vi "theremin.vi"() -> ()   [LabVIEW 2024]
uses:
  <vilib>/Instr/_visa.llb/VISA Configure Serial Port (Instr).vi
panel:
  out "STANDBY":bool
  out "G#":bool
  out "G":bool
  out "F#":bool
  out "F":bool
  out "E":bool
  out "D#":bool
  out "D":bool
  out "C#":bool
  out "C":bool
  out "B":bool
  out "A#":bool
  out "A":bool
  out "Octave 8":bool
  out "Octave 7":bool
  out "Octave 6":bool
  out "Octave 5":bool
  out "Octave 4":bool
  out "Octave 3":bool
  out "Octave 2":bool
  out "Octave 1":bool
  out "Octave 0":bool
  out "Frequency":dbl
  in  "stop":bool
  out "Volume":dbl(knob) scale=0.0..255.0
  out "Pitch":dbl(knob) scale=0.0..1000.0
  in  "VISA resource name":refnum<visa-resource-name>
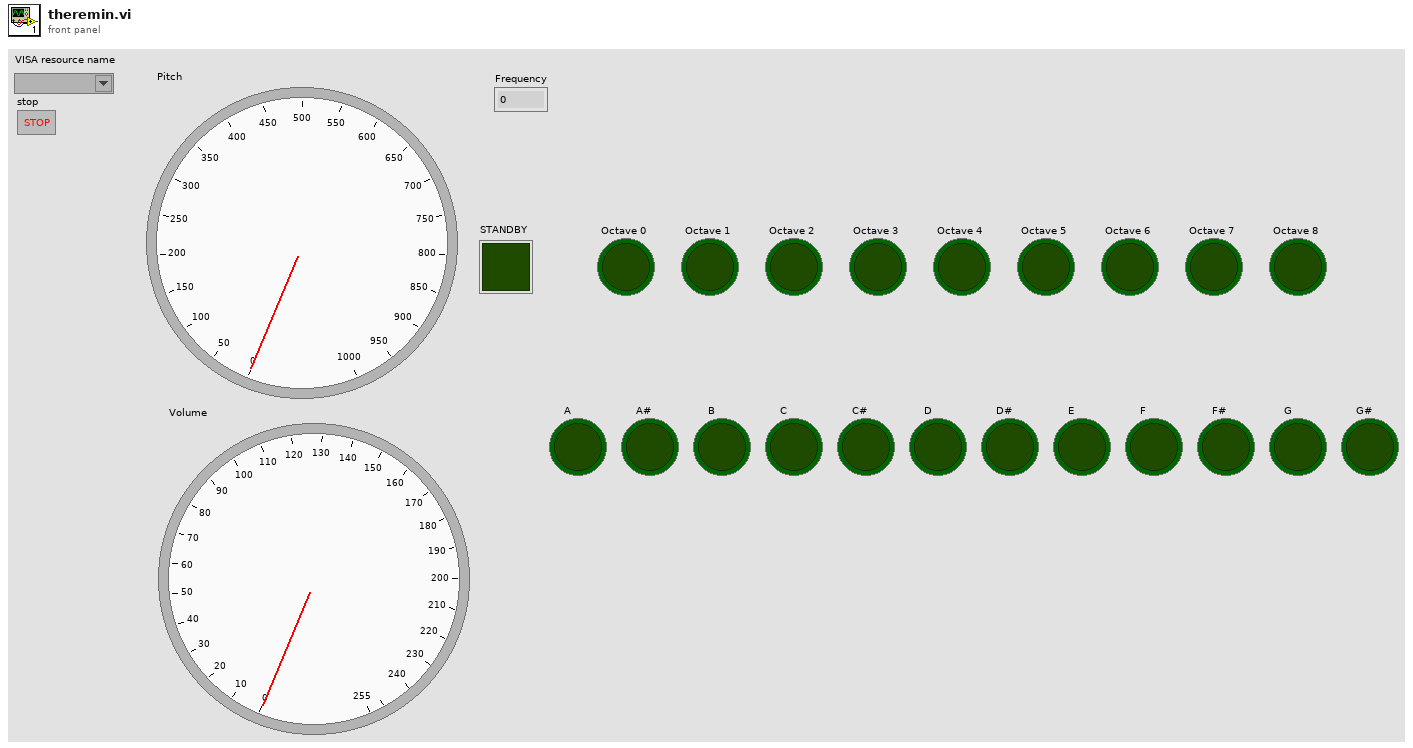
[diagram p1: front panel]
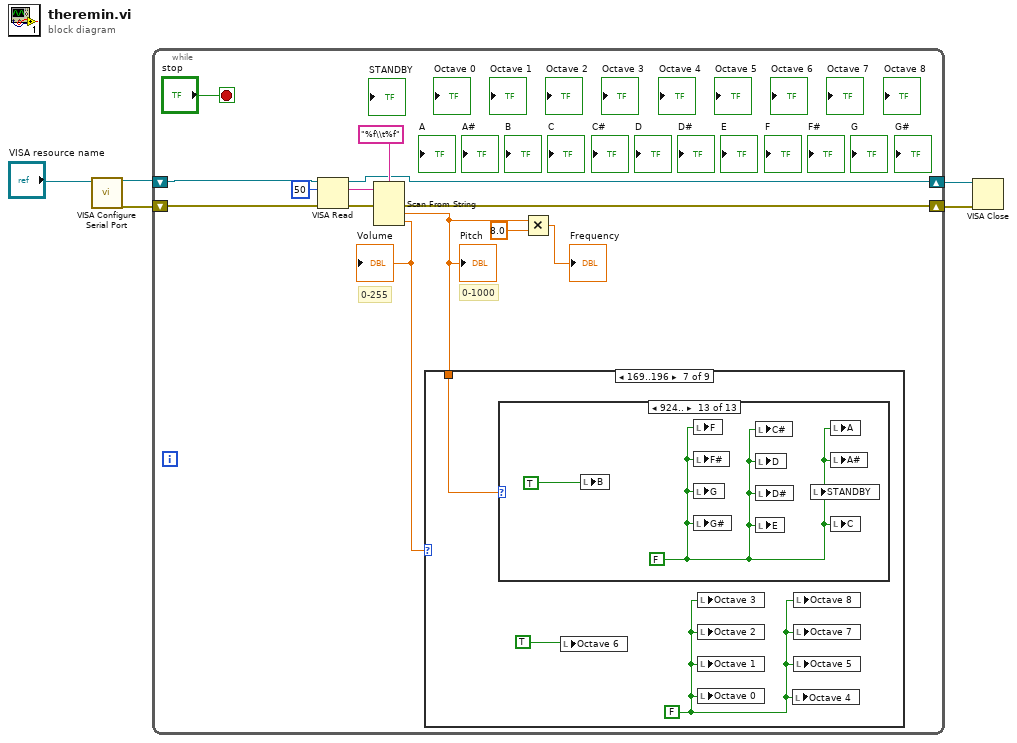
[diagram p0: block diagram]
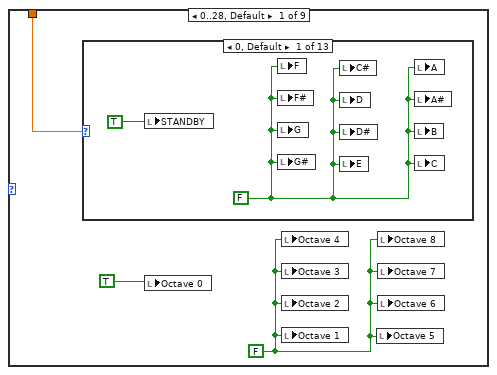
[diagram p2: hidden frame]
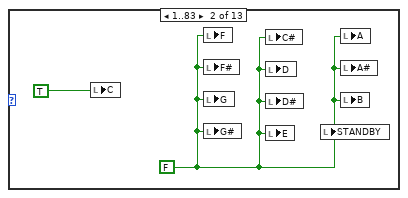
[diagram p3: hidden frame]
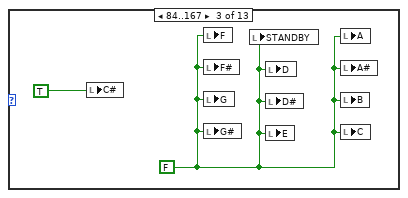
[diagram p4: hidden frame]
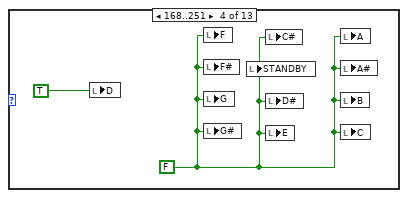
[diagram p5: hidden frame]
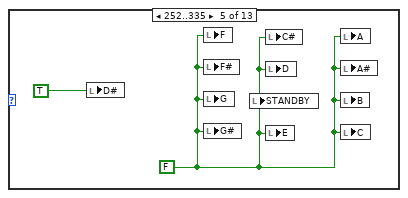
[diagram p6: hidden frame]
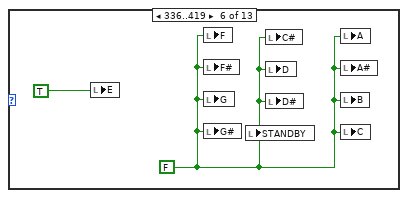
[diagram p7: hidden frame]
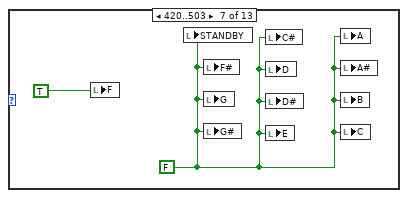
[diagram p8: hidden frame]
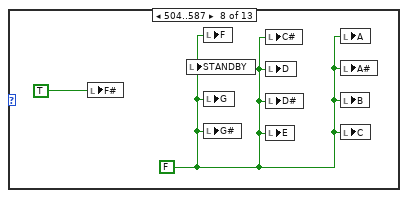
[diagram p9: hidden frame]
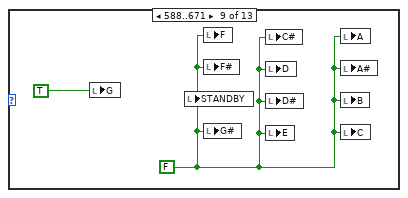
[diagram p10: hidden frame]
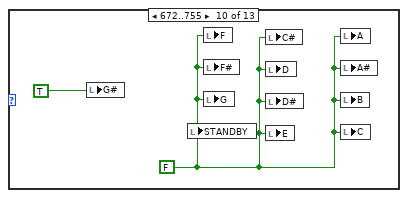
[diagram p11: hidden frame]
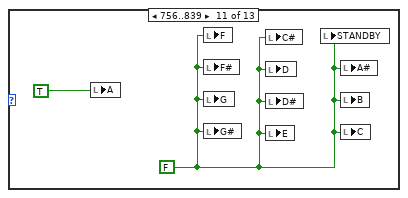
[diagram p12: hidden frame]
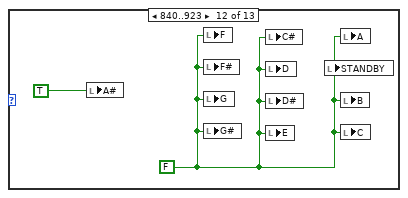
[diagram p13: hidden frame]
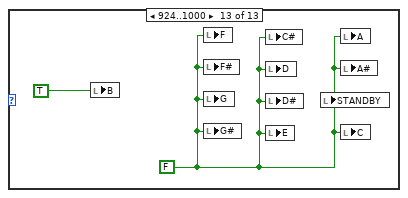
[diagram p14: hidden frame]
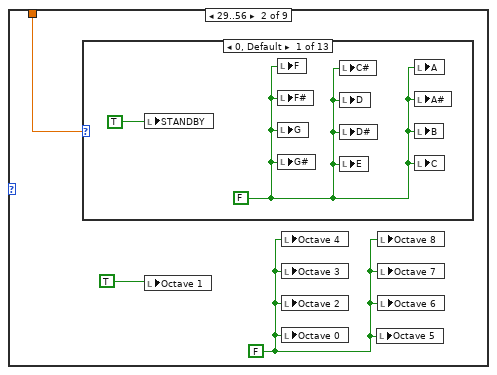
[diagram p15: hidden frame]
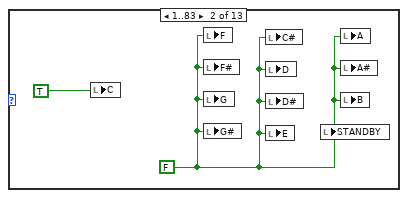
[diagram p16: hidden frame]
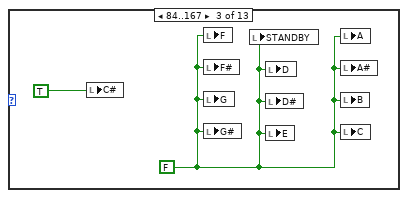
[diagram p17: hidden frame]
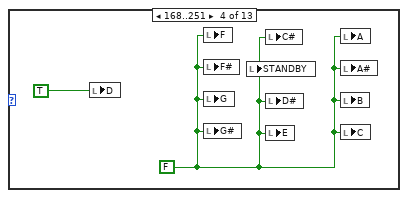
[diagram p18: hidden frame]
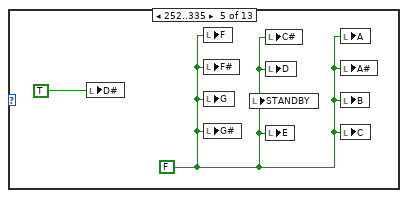
[diagram p19: hidden frame]
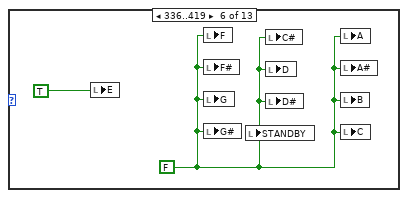
[diagram p20: hidden frame]
diagram:
  n1 = call-poly "VISA Configure Serial Port"("VISA resource name"="VISA resource name") -> ("VISA resource name out"=w3:refnum<visa-resource-name>, "error out"=w2:errorcluster)  [unwired: 13 in]
  n2 = while {
    shift-right: [w15] -> w4
    shift-left: w3 -> [w12]
    shift-right: [w18] -> w5
    shift-left: w2 -> [w13]
    stop <- "stop" stop-if-true
    # "0-1000"
    # "0-255"
    n3 = VISA Read(VISA resource name=w12, byte count=u32 50, error in (no error)=w13) -> (VISA resource name out=w15:refnum<visa-resource-name>, read buffer=w10:string, error out=w14:errorcluster)  [unwired: 1 out]
    n4 = Scan From String(format string="%f\\t%f", input string=w10, error in=w14) -> (error out=w18:errorcluster, output 1=w7:dbl, output 2=w6:dbl)  [unwired: 3 in, 2 out]
    "Pitch" <- w7
    "Volume" <- w6
    n5 = case shown="169..196" w6 {
      tunnel: w7 -> [w21 w50 w79 w108 w137 w166 w195 w224 w253]
      frame 0..28, Default {
        w19 = FALSE
        n6 = case shown="0, Default" w21 {
          frame 0, Default {
            w22 = FALSE
            n7 = local write "STANDBY"(TRUE) -> ()
            n8 = local write "F"(w22) -> ()
            n9 = local write "F#"(w22) -> ()
            n10 = local write "G"(w22) -> ()
            n11 = local write "G#"(w22) -> ()
            n12 = local write "C#"(w22) -> ()
            n13 = local write "D"(w22) -> ()
            n14 = local write "D#"(w22) -> ()
            n15 = local write "E"(w22) -> ()
            n16 = local write "A"(w22) -> ()
            n17 = local write "A#"(w22) -> ()
            n18 = local write "B"(w22) -> ()
            n19 = local write "C"(w22) -> ()
          }
          frame 1..83 {
            w24 = FALSE
            n20 = local write "C"(TRUE) -> ()
            n21 = local write "F"(w24) -> ()
            n22 = local write "F#"(w24) -> ()
            n23 = local write "G"(w24) -> ()
            n24 = local write "G#"(w24) -> ()
            n25 = local write "C#"(w24) -> ()
            n26 = local write "D"(w24) -> ()
            n27 = local write "D#"(w24) -> ()
            n28 = local write "E"(w24) -> ()
            n29 = local write "STANDBY"(w24) -> ()
            n30 = local write "A"(w24) -> ()
            n31 = local write "A#"(w24) -> ()
            n32 = local write "B"(w24) -> ()
          }
          frame 84..167 {
            w26 = FALSE
            n33 = local write "C#"(TRUE) -> ()
            n34 = local write "F"(w26) -> ()
            n35 = local write "F#"(w26) -> ()
            n36 = local write "G"(w26) -> ()
            n37 = local write "G#"(w26) -> ()
            n38 = local write "STANDBY"(w26) -> ()
            n39 = local write "D"(w26) -> ()
            n40 = local write "D#"(w26) -> ()
            n41 = local write "E"(w26) -> ()
            n42 = local write "A"(w26) -> ()
            n43 = local write "A#"(w26) -> ()
            n44 = local write "B"(w26) -> ()
            n45 = local write "C"(w26) -> ()
          }
          frame 168..251 {
            w28 = FALSE
            n46 = local write "D"(TRUE) -> ()
            n47 = local write "F"(w28) -> ()
            n48 = local write "F#"(w28) -> ()
            n49 = local write "G"(w28) -> ()
            n50 = local write "G#"(w28) -> ()
            n51 = local write "STANDBY"(w28) -> ()
            n52 = local write "C#"(w28) -> ()
            n53 = local write "D#"(w28) -> ()
            n54 = local write "E"(w28) -> ()
            n55 = local write "A"(w28) -> ()
            n56 = local write "A#"(w28) -> ()
            n57 = local write "B"(w28) -> ()
            n58 = local write "C"(w28) -> ()
          }
          frame 252..335 {
            w30 = FALSE
            n59 = local write "D#"(TRUE) -> ()
            n60 = local write "F"(w30) -> ()
            n61 = local write "F#"(w30) -> ()
            n62 = local write "G"(w30) -> ()
            n63 = local write "G#"(w30) -> ()
            n64 = local write "STANDBY"(w30) -> ()
            n65 = local write "C#"(w30) -> ()
            n66 = local write "D"(w30) -> ()
            n67 = local write "E"(w30) -> ()
            n68 = local write "A"(w30) -> ()
            n69 = local write "A#"(w30) -> ()
            n70 = local write "B"(w30) -> ()
            n71 = local write "C"(w30) -> ()
          }
          frame 336..419 {
            w32 = FALSE
            n72 = local write "E"(TRUE) -> ()
            n73 = local write "F"(w32) -> ()
            n74 = local write "F#"(w32) -> ()
            n75 = local write "G"(w32) -> ()
            n76 = local write "G#"(w32) -> ()
            n77 = local write "STANDBY"(w32) -> ()
            n78 = local write "C#"(w32) -> ()
            n79 = local write "D"(w32) -> ()
            n80 = local write "D#"(w32) -> ()
            n81 = local write "A"(w32) -> ()
            n82 = local write "A#"(w32) -> ()
            n83 = local write "B"(w32) -> ()
            n84 = local write "C"(w32) -> ()
          }
          frame 420..503 {
            w34 = FALSE
            n85 = local write "F"(TRUE) -> ()
            n86 = local write "STANDBY"(w34) -> ()
            n87 = local write "F#"(w34) -> ()
            n88 = local write "G"(w34) -> ()
            n89 = local write "G#"(w34) -> ()
            n90 = local write "C#"(w34) -> ()
            n91 = local write "D"(w34) -> ()
            n92 = local write "D#"(w34) -> ()
            n93 = local write "E"(w34) -> ()
            n94 = local write "A"(w34) -> ()
            n95 = local write "A#"(w34) -> ()
            n96 = local write "B"(w34) -> ()
            n97 = local write "C"(w34) -> ()
          }
          frame 504..587 {
            w36 = FALSE
            n98 = local write "F#"(TRUE) -> ()
            n99 = local write "STANDBY"(w36) -> ()
            n100 = local write "F"(w36) -> ()
            n101 = local write "G"(w36) -> ()
            n102 = local write "G#"(w36) -> ()
            n103 = local write "C#"(w36) -> ()
            n104 = local write "D"(w36) -> ()
            n105 = local write "D#"(w36) -> ()
            n106 = local write "E"(w36) -> ()
            n107 = local write "A"(w36) -> ()
            n108 = local write "A#"(w36) -> ()
            n109 = local write "B"(w36) -> ()
            n110 = local write "C"(w36) -> ()
          }
          frame 588..671 {
            w38 = FALSE
            n111 = local write "G"(TRUE) -> ()
            n112 = local write "STANDBY"(w38) -> ()
            n113 = local write "F"(w38) -> ()
            n114 = local write "F#"(w38) -> ()
            n115 = local write "G#"(w38) -> ()
            n116 = local write "C#"(w38) -> ()
            n117 = local write "D"(w38) -> ()
            n118 = local write "D#"(w38) -> ()
            n119 = local write "E"(w38) -> ()
            n120 = local write "A"(w38) -> ()
            n121 = local write "A#"(w38) -> ()
            n122 = local write "B"(w38) -> ()
            n123 = local write "C"(w38) -> ()
          }
          frame 672..755 {
            w40 = FALSE
            n124 = local write "G#"(TRUE) -> ()
            n125 = local write "STANDBY"(w40) -> ()
            n126 = local write "F"(w40) -> ()
            n127 = local write "F#"(w40) -> ()
            n128 = local write "G"(w40) -> ()
            n129 = local write "C#"(w40) -> ()
            n130 = local write "D"(w40) -> ()
            n131 = local write "D#"(w40) -> ()
            n132 = local write "E"(w40) -> ()
            n133 = local write "A"(w40) -> ()
            n134 = local write "A#"(w40) -> ()
            n135 = local write "B"(w40) -> ()
            n136 = local write "C"(w40) -> ()
          }
          frame 756..839 {
            w42 = FALSE
            n137 = local write "A"(TRUE) -> ()
            n138 = local write "F"(w42) -> ()
            n139 = local write "F#"(w42) -> ()
            n140 = local write "G"(w42) -> ()
            n141 = local write "G#"(w42) -> ()
            n142 = local write "C#"(w42) -> ()
            n143 = local write "D"(w42) -> ()
            n144 = local write "D#"(w42) -> ()
            n145 = local write "E"(w42) -> ()
            n146 = local write "STANDBY"(w42) -> ()
            n147 = local write "A#"(w42) -> ()
            n148 = local write "B"(w42) -> ()
            n149 = local write "C"(w42) -> ()
          }
          frame 840..923 {
            w44 = FALSE
            n150 = local write "A#"(TRUE) -> ()
            n151 = local write "F"(w44) -> ()
            n152 = local write "F#"(w44) -> ()
            n153 = local write "G"(w44) -> ()
            n154 = local write "G#"(w44) -> ()
            n155 = local write "C#"(w44) -> ()
            n156 = local write "D"(w44) -> ()
            n157 = local write "D#"(w44) -> ()
            n158 = local write "E"(w44) -> ()
            n159 = local write "STANDBY"(w44) -> ()
            n160 = local write "A"(w44) -> ()
            n161 = local write "B"(w44) -> ()
            n162 = local write "C"(w44) -> ()
          }
          frame 924..1000 {
            w46 = FALSE
            n163 = local write "B"(TRUE) -> ()
            n164 = local write "F"(w46) -> ()
            n165 = local write "F#"(w46) -> ()
            n166 = local write "G"(w46) -> ()
            n167 = local write "G#"(w46) -> ()
            n168 = local write "C#"(w46) -> ()
            n169 = local write "D"(w46) -> ()
            n170 = local write "D#"(w46) -> ()
            n171 = local write "E"(w46) -> ()
            n172 = local write "STANDBY"(w46) -> ()
            n173 = local write "A"(w46) -> ()
            n174 = local write "A#"(w46) -> ()
            n175 = local write "C"(w46) -> ()
          }
        }
        n176 = local write "Octave 0"(TRUE) -> ()
        n177 = local write "Octave 4"(w19) -> ()
        n178 = local write "Octave 3"(w19) -> ()
        n179 = local write "Octave 2"(w19) -> ()
        n180 = local write "Octave 1"(w19) -> ()
        n181 = local write "Octave 5"(w19) -> ()
        n182 = local write "Octave 8"(w19) -> ()
        n183 = local write "Octave 7"(w19) -> ()
        n184 = local write "Octave 6"(w19) -> ()
      }
      frame 29..56 {
        w48 = FALSE
        n185 = case shown="0, Default" w50 {
          frame 0, Default {
            w51 = FALSE
            n186 = local write "STANDBY"(TRUE) -> ()
            n187 = local write "F"(w51) -> ()
            n188 = local write "F#"(w51) -> ()
            n189 = local write "G"(w51) -> ()
            n190 = local write "G#"(w51) -> ()
            n191 = local write "C#"(w51) -> ()
            n192 = local write "D"(w51) -> ()
            n193 = local write "D#"(w51) -> ()
            n194 = local write "E"(w51) -> ()
            n195 = local write "A"(w51) -> ()
            n196 = local write "A#"(w51) -> ()
            n197 = local write "B"(w51) -> ()
            n198 = local write "C"(w51) -> ()
          }
          frame 1..83 {
            w53 = FALSE
            n199 = local write "C"(TRUE) -> ()
            n200 = local write "F"(w53) -> ()
            n201 = local write "F#"(w53) -> ()
            n202 = local write "G"(w53) -> ()
            n203 = local write "G#"(w53) -> ()
            n204 = local write "C#"(w53) -> ()
            n205 = local write "D"(w53) -> ()
            n206 = local write "D#"(w53) -> ()
            n207 = local write "E"(w53) -> ()
            n208 = local write "STANDBY"(w53) -> ()
            n209 = local write "A"(w53) -> ()
            n210 = local write "A#"(w53) -> ()
            n211 = local write "B"(w53) -> ()
          }
          frame 84..167 {
            w55 = FALSE
            n212 = local write "C#"(TRUE) -> ()
            n213 = local write "F"(w55) -> ()
            n214 = local write "F#"(w55) -> ()
            n215 = local write "G"(w55) -> ()
            n216 = local write "G#"(w55) -> ()
            n217 = local write "STANDBY"(w55) -> ()
            n218 = local write "D"(w55) -> ()
            n219 = local write "D#"(w55) -> ()
            n220 = local write "E"(w55) -> ()
            n221 = local write "A"(w55) -> ()
            n222 = local write "A#"(w55) -> ()
            n223 = local write "B"(w55) -> ()
            n224 = local write "C"(w55) -> ()
          }
          frame 168..251 {
            w57 = FALSE
            n225 = local write "D"(TRUE) -> ()
            n226 = local write "F"(w57) -> ()
            n227 = local write "F#"(w57) -> ()
            n228 = local write "G"(w57) -> ()
            n229 = local write "G#"(w57) -> ()
            n230 = local write "STANDBY"(w57) -> ()
            n231 = local write "C#"(w57) -> ()
            n232 = local write "D#"(w57) -> ()
            n233 = local write "E"(w57) -> ()
            n234 = local write "A"(w57) -> ()
            n235 = local write "A#"(w57) -> ()
            n236 = local write "B"(w57) -> ()
            n237 = local write "C"(w57) -> ()
          }
          frame 252..335 {
            w59 = FALSE
            n238 = local write "D#"(TRUE) -> ()
            n239 = local write "F"(w59) -> ()
            n240 = local write "F#"(w59) -> ()
            n241 = local write "G"(w59) -> ()
            n242 = local write "G#"(w59) -> ()
            n243 = local write "STANDBY"(w59) -> ()
            n244 = local write "C#"(w59) -> ()
            n245 = local write "D"(w59) -> ()
            n246 = local write "E"(w59) -> ()
            n247 = local write "A"(w59) -> ()
            n248 = local write "A#"(w59) -> ()
            n249 = local write "B"(w59) -> ()
            n250 = local write "C"(w59) -> ()
          }
          frame 336..419 {
            w61 = FALSE
            n251 = local write "E"(TRUE) -> ()
            n252 = local write "F"(w61) -> ()
            n253 = local write "F#"(w61) -> ()
            n254 = local write "G"(w61) -> ()
            n255 = local write "G#"(w61) -> ()
            n256 = local write "STANDBY"(w61) -> ()
            n257 = local write "C#"(w61) -> ()
            n258 = local write "D"(w61) -> ()
            n259 = local write "D#"(w61) -> ()
            n260 = local write "A"(w61) -> ()
            n261 = local write "A#"(w61) -> ()
            n262 = local write "B"(w61) -> ()
            n263 = local write "C"(w61) -> ()
          }
          frame 420..503 {
            w63 = FALSE
            n264 = local write "F"(TRUE) -> ()
            n265 = local write "STANDBY"(w63) -> ()
            n266 = local write "F#"(w63) -> ()
            n267 = local write "G"(w63) -> ()
            n268 = local write "G#"(w63) -> ()
            n269 = local write "C#"(w63) -> ()
            n270 = local write "D"(w63) -> ()
            n271 = local write "D#"(w63) -> ()
            n272 = local write "E"(w63) -> ()
            n273 = local write "A"(w63) -> ()
            n274 = local write "A#"(w63) -> ()
            n275 = local write "B"(w63) -> ()
            n276 = local write "C"(w63) -> ()
          }
          frame 504..587 {
            w65 = FALSE
            n277 = local write "F#"(TRUE) -> ()
            n278 = local write "STANDBY"(w65) -> ()
            n279 = local write "F"(w65) -> ()
            n280 = local write "G"(w65) -> ()
            n281 = local write "G#"(w65) -> ()
            n282 = local write "C#"(w65) -> ()
            n283 = local write "D"(w65) -> ()
            n284 = local write "D#"(w65) -> ()
            n285 = local write "E"(w65) -> ()
            n286 = local write "A"(w65) -> ()
            n287 = local write "A#"(w65) -> ()
            n288 = local write "B"(w65) -> ()
            n289 = local write "C"(w65) -> ()
          }
          frame 588..671 {
            w67 = FALSE
            n290 = local write "G"(TRUE) -> ()
            n291 = local write "STANDBY"(w67) -> ()
            n292 = local write "F"(w67) -> ()
            n293 = local write "F#"(w67) -> ()
            n294 = local write "G#"(w67) -> ()
            n295 = local write "C#"(w67) -> ()
            n296 = local write "D"(w67) -> ()
            n297 = local write "D#"(w67) -> ()
            n298 = local write "E"(w67) -> ()
            n299 = local write "A"(w67) -> ()
            n300 = local write "A#"(w67) -> ()
            n301 = local write "B"(w67) -> ()
            n302 = local write "C"(w67) -> ()
          }
          frame 672..755 {
            w69 = FALSE
            n303 = local write "G#"(TRUE) -> ()
            n304 = local write "STANDBY"(w69) -> ()
            n305 = local write "F"(w69) -> ()
            n306 = local write "F#"(w69) -> ()
            n307 = local write "G"(w69) -> ()
            n308 = local write "C#"(w69) -> ()
            n309 = local write "D"(w69) -> ()
            n310 = local write "D#"(w69) -> ()
            n311 = local write "E"(w69) -> ()
            n312 = local write "A"(w69) -> ()
            n313 = local write "A#"(w69) -> ()
            n314 = local write "B"(w69) -> ()
            n315 = local write "C"(w69) -> ()
          }
          frame 756..839 {
            w71 = FALSE
            n316 = local write "A"(TRUE) -> ()
            n317 = local write "F"(w71) -> ()
            n318 = local write "F#"(w71) -> ()
            n319 = local write "G"(w71) -> ()
            n320 = local write "G#"(w71) -> ()
            n321 = local write "C#"(w71) -> ()
            n322 = local write "D"(w71) -> ()
            n323 = local write "D#"(w71) -> ()
            n324 = local write "E"(w71) -> ()
            n325 = local write "STANDBY"(w71) -> ()
            n326 = local write "A#"(w71) -> ()
            n327 = local write "B"(w71) -> ()
            n328 = local write "C"(w71) -> ()
          }
          frame 840..923 {
            w73 = FALSE
            n329 = local write "A#"(TRUE) -> ()
            n330 = local write "F"(w73) -> ()
            n331 = local write "F#"(w73) -> ()
            n332 = local write "G"(w73) -> ()
            n333 = local write "G#"(w73) -> ()
            n334 = local write "C#"(w73) -> ()
            n335 = local write "D"(w73) -> ()
            n336 = local write "D#"(w73) -> ()
            n337 = local write "E"(w73) -> ()
            n338 = local write "STANDBY"(w73) -> ()
            n339 = local write "A"(w73) -> ()
            n340 = local write "B"(w73) -> ()
            n341 = local write "C"(w73) -> ()
          }
          frame 924..1000 {
            w75 = FALSE
            n342 = local write "B"(TRUE) -> ()
            n343 = local write "F"(w75) -> ()
            n344 = local write "F#"(w75) -> ()
            n345 = local write "G"(w75) -> ()
            n346 = local write "G#"(w75) -> ()
            n347 = local write "C#"(w75) -> ()
            n348 = local write "D"(w75) -> ()
            n349 = local write "D#"(w75) -> ()
            n350 = local write "E"(w75) -> ()
            n351 = local write "STANDBY"(w75) -> ()
            n352 = local write "A"(w75) -> ()
            n353 = local write "A#"(w75) -> ()
            n354 = local write "C"(w75) -> ()
          }
        }
        n355 = local write "Octave 1"(TRUE) -> ()
        n356 = local write "Octave 4"(w48) -> ()
        n357 = local write "Octave 3"(w48) -> ()
        n358 = local write "Octave 2"(w48) -> ()
        n359 = local write "Octave 0"(w48) -> ()
        n360 = local write "Octave 5"(w48) -> ()
        n361 = local write "Octave 8"(w48) -> ()
        n362 = local write "Octave 7"(w48) -> ()
        n363 = local write "Octave 6"(w48) -> ()
      }
      frame 57..84 {
        w77 = FALSE
        n364 = case shown="0, Default" w79 {
          frame 0, Default {
            w80 = FALSE
            n365 = local write "STANDBY"(TRUE) -> ()
            n366 = local write "F"(w80) -> ()
            n367 = local write "F#"(w80) -> ()
            n368 = local write "G"(w80) -> ()
            n369 = local write "G#"(w80) -> ()
            n370 = local write "C#"(w80) -> ()
            n371 = local write "D"(w80) -> ()
            n372 = local write "D#"(w80) -> ()
            n373 = local write "E"(w80) -> ()
            n374 = local write "A"(w80) -> ()
            n375 = local write "A#"(w80) -> ()
            n376 = local write "B"(w80) -> ()
            n377 = local write "C"(w80) -> ()
          }
          frame 1..83 {
            w82 = FALSE
            n378 = local write "C"(TRUE) -> ()
            n379 = local write "F"(w82) -> ()
            n380 = local write "F#"(w82) -> ()
            n381 = local write "G"(w82) -> ()
            n382 = local write "G#"(w82) -> ()
            n383 = local write "C#"(w82) -> ()
            n384 = local write "D"(w82) -> ()
            n385 = local write "D#"(w82) -> ()
            n386 = local write "E"(w82) -> ()
            n387 = local write "STANDBY"(w82) -> ()
            n388 = local write "A"(w82) -> ()
            n389 = local write "A#"(w82) -> ()
            n390 = local write "B"(w82) -> ()
          }
          frame 84..167 {
            w84 = FALSE
            n391 = local write "C#"(TRUE) -> ()
            n392 = local write "F"(w84) -> ()
            n393 = local write "F#"(w84) -> ()
            n394 = local write "G"(w84) -> ()
            n395 = local write "G#"(w84) -> ()
            n396 = local write "STANDBY"(w84) -> ()
            n397 = local write "D"(w84) -> ()
            n398 = local write "D#"(w84) -> ()
            n399 = local write "E"(w84) -> ()
            n400 = local write "A"(w84) -> ()
            n401 = local write "A#"(w84) -> ()
            n402 = local write "B"(w84) -> ()
            n403 = local write "C"(w84) -> ()
          }
          frame 168..251 {
            w86 = FALSE
            n404 = local write "D"(TRUE) -> ()
            n405 = local write "F"(w86) -> ()
            n406 = local write "F#"(w86) -> ()
            n407 = local write "G"(w86) -> ()
            n408 = local write "G#"(w86) -> ()
            n409 = local write "STANDBY"(w86) -> ()
            n410 = local write "C#"(w86) -> ()
            n411 = local write "D#"(w86) -> ()
            n412 = local write "E"(w86) -> ()
            n413 = local write "A"(w86) -> ()
            n414 = local write "A#"(w86) -> ()
            n415 = local write "B"(w86) -> ()
            n416 = local write "C"(w86) -> ()
          }
          frame 252..335 {
            w88 = FALSE
            n417 = local write "D#"(TRUE) -> ()
            n418 = local write "F"(w88) -> ()
            n419 = local write "F#"(w88) -> ()
            n420 = local write "G"(w88) -> ()
            n421 = local write "G#"(w88) -> ()
            n422 = local write "STANDBY"(w88) -> ()
            n423 = local write "C#"(w88) -> ()
            n424 = local write "D"(w88) -> ()
            n425 = local write "E"(w88) -> ()
            n426 = local write "A"(w88) -> ()
            n427 = local write "A#"(w88) -> ()
            n428 = local write "B"(w88) -> ()
            n429 = local write "C"(w88) -> ()
          }
          frame 336..419 {
            w90 = FALSE
            n430 = local write "E"(TRUE) -> ()
            n431 = local write "F"(w90) -> ()
            n432 = local write "F#"(w90) -> ()
            n433 = local write "G"(w90) -> ()
            n434 = local write "G#"(w90) -> ()
            n435 = local write "STANDBY"(w90) -> ()
            n436 = local write "C#"(w90) -> ()
            n437 = local write "D"(w90) -> ()
            n438 = local write "D#"(w90) -> ()
            n439 = local write "A"(w90) -> ()
            n440 = local write "A#"(w90) -> ()
            n441 = local write "B"(w90) -> ()
            n442 = local write "C"(w90) -> ()
          }
          frame 420..503 {
            w92 = FALSE
            n443 = local write "F"(TRUE) -> ()
            n444 = local write "STANDBY"(w92) -> ()
            n445 = local write "F#"(w92) -> ()
            n446 = local write "G"(w92) -> ()
            n447 = local write "G#"(w92) -> ()
            n448 = local write "C#"(w92) -> ()
            n449 = local write "D"(w92) -> ()
            n450 = local write "D#"(w92) -> ()
            n451 = local write "E"(w92) -> ()
            n452 = local write "A"(w92) -> ()
            n453 = local write "A#"(w92) -> ()
            n454 = local write "B"(w92) -> ()
            n455 = local write "C"(w92) -> ()
          }
          frame 504..587 {
            w94 = FALSE
            n456 = local write "F#"(TRUE) -> ()
            n457 = local write "STANDBY"(w94) -> ()
            n458 = local write "F"(w94) -> ()
            n459 = local write "G"(w94) -> ()
            n460 = local write "G#"(w94) -> ()
            n461 = local write "C#"(w94) -> ()
            n462 = local write "D"(w94) -> ()
            n463 = local write "D#"(w94) -> ()
            n464 = local write "E"(w94) -> ()
            n465 = local write "A"(w94) -> ()
            n466 = local write "A#"(w94) -> ()
            n467 = local write "B"(w94) -> ()
            n468 = local write "C"(w94) -> ()
          }
          frame 588..671 {
            w96 = FALSE
            n469 = local write "G"(TRUE) -> ()
            n470 = local write "STANDBY"(w96) -> ()
            n471 = local write "F"(w96) -> ()
            n472 = local write "F#"(w96) -> ()
            n473 = local write "G#"(w96) -> ()
            n474 = local write "C#"(w96) -> ()
            n475 = local write "D"(w96) -> ()
            n476 = local write "D#"(w96) -> ()
            n477 = local write "E"(w96) -> ()
            n478 = local write "A"(w96) -> ()
            n479 = local write "A#"(w96) -> ()
            n480 = local write "B"(w96) -> ()
            n481 = local write "C"(w96) -> ()
          }
          frame 672..755 {
            w98 = FALSE
            n482 = local write "G#"(TRUE) -> ()
            n483 = local write "STANDBY"(w98) -> ()
            n484 = local write "F"(w98) -> ()
            n485 = local write "F#"(w98) -> ()
            n486 = local write "G"(w98) -> ()
            n487 = local write "C#"(w98) -> ()
            n488 = local write "D"(w98) -> ()
            n489 = local write "D#"(w98) -> ()
            n490 = local write "E"(w98) -> ()
            n491 = local write "A"(w98) -> ()
            n492 = local write "A#"(w98) -> ()
            n493 = local write "B"(w98) -> ()
            n494 = local write "C"(w98) -> ()
          }
          frame 756..839 {
            w100 = FALSE
            n495 = local write "A"(TRUE) -> ()
            n496 = local write "F"(w100) -> ()
            n497 = local write "F#"(w100) -> ()
            n498 = local write "G"(w100) -> ()
            n499 = local write "G#"(w100) -> ()
            n500 = local write "C#"(w100) -> ()
            n501 = local write "D"(w100) -> ()
            n502 = local write "D#"(w100) -> ()
            n503 = local write "E"(w100) -> ()
            n504 = local write "STANDBY"(w100) -> ()
            n505 = local write "A#"(w100) -> ()
            n506 = local write "B"(w100) -> ()
            n507 = local write "C"(w100) -> ()
          }
          frame 840..923 {
            w102 = FALSE
            n508 = local write "A#"(TRUE) -> ()
            n509 = local write "F"(w102) -> ()
            n510 = local write "F#"(w102) -> ()
            n511 = local write "G"(w102) -> ()
            n512 = local write "G#"(w102) -> ()
            n513 = local write "C#"(w102) -> ()
            n514 = local write "D"(w102) -> ()
            n515 = local write "D#"(w102) -> ()
            n516 = local write "E"(w102) -> ()
            n517 = local write "STANDBY"(w102) -> ()
            n518 = local write "A"(w102) -> ()
            n519 = local write "B"(w102) -> ()
            n520 = local write "C"(w102) -> ()
          }
          frame 924..1000 {
            w104 = FALSE
            n521 = local write "B"(TRUE) -> ()
            n522 = local write "F"(w104) -> ()
            n523 = local write "F#"(w104) -> ()
            n524 = local write "G"(w104) -> ()
            n525 = local write "G#"(w104) -> ()
            n526 = local write "C#"(w104) -> ()
            n527 = local write "D"(w104) -> ()
            n528 = local write "D#"(w104) -> ()
            n529 = local write "E"(w104) -> ()
            n530 = local write "STANDBY"(w104) -> ()
            n531 = local write "A"(w104) -> ()
            n532 = local write "A#"(w104) -> ()
            n533 = local write "C"(w104) -> ()
          }
        }
        n534 = local write "Octave 2"(TRUE) -> ()
        n535 = local write "Octave 4"(w77) -> ()
        n536 = local write "Octave 3"(w77) -> ()
        n537 = local write "Octave 1"(w77) -> ()
        n538 = local write "Octave 0"(w77) -> ()
        n539 = local write "Octave 5"(w77) -> ()
        n540 = local write "Octave 8"(w77) -> ()
        n541 = local write "Octave 7"(w77) -> ()
        n542 = local write "Octave 6"(w77) -> ()
      }
      frame 85..112 {
        w106 = FALSE
        n543 = case shown="0, Default" w108 {
          frame 0, Default {
            w109 = FALSE
            n544 = local write "STANDBY"(TRUE) -> ()
            n545 = local write "F"(w109) -> ()
            n546 = local write "F#"(w109) -> ()
            n547 = local write "G"(w109) -> ()
            n548 = local write "G#"(w109) -> ()
            n549 = local write "C#"(w109) -> ()
            n550 = local write "D"(w109) -> ()
            n551 = local write "D#"(w109) -> ()
            n552 = local write "E"(w109) -> ()
            n553 = local write "A"(w109) -> ()
            n554 = local write "A#"(w109) -> ()
            n555 = local write "B"(w109) -> ()
            n556 = local write "C"(w109) -> ()
          }
          frame 1..83 {
            w111 = FALSE
            n557 = local write "C"(TRUE) -> ()
            n558 = local write "F"(w111) -> ()
            n559 = local write "F#"(w111) -> ()
            n560 = local write "G"(w111) -> ()
            n561 = local write "G#"(w111) -> ()
            n562 = local write "C#"(w111) -> ()
            n563 = local write "D"(w111) -> ()
            n564 = local write "D#"(w111) -> ()
            n565 = local write "E"(w111) -> ()
            n566 = local write "STANDBY"(w111) -> ()
            n567 = local write "A"(w111) -> ()
            n568 = local write "A#"(w111) -> ()
            n569 = local write "B"(w111) -> ()
          }
          frame 84..167 {
            w113 = FALSE
            n570 = local write "C#"(TRUE) -> ()
            n571 = local write "F"(w113) -> ()
            n572 = local write "F#"(w113) -> ()
            n573 = local write "G"(w113) -> ()
            n574 = local write "G#"(w113) -> ()
            n575 = local write "STANDBY"(w113) -> ()
            n576 = local write "D"(w113) -> ()
            n577 = local write "D#"(w113) -> ()
            n578 = local write "E"(w113) -> ()
            n579 = local write "A"(w113) -> ()
            n580 = local write "A#"(w113) -> ()
            n581 = local write "B"(w113) -> ()
            n582 = local write "C"(w113) -> ()
          }
          frame 168..251 {
            w115 = FALSE
            n583 = local write "D"(TRUE) -> ()
            n584 = local write "F"(w115) -> ()
            n585 = local write "F#"(w115) -> ()
            n586 = local write "G"(w115) -> ()
            n587 = local write "G#"(w115) -> ()
            n588 = local write "STANDBY"(w115) -> ()
            n589 = local write "C#"(w115) -> ()
            n590 = local write "D#"(w115) -> ()
            n591 = local write "E"(w115) -> ()
            n592 = local write "A"(w115) -> ()
            n593 = local write "A#"(w115) -> ()
            n594 = local write "B"(w115) -> ()
            n595 = local write "C"(w115) -> ()
          }
          frame 252..335 {
            w117 = FALSE
            n596 = local write "D#"(TRUE) -> ()
            n597 = local write "F"(w117) -> ()
            n598 = local write "F#"(w117) -> ()
            n599 = local write "G"(w117) -> ()
            n600 = local write "G#"(w117) -> ()
            n601 = local write "STANDBY"(w117) -> ()
            n602 = local write "C#"(w117) -> ()
            n603 = local write "D"(w117) -> ()
            n604 = local write "E"(w117) -> ()
            n605 = local write "A"(w117) -> ()
            n606 = local write "A#"(w117) -> ()
            n607 = local write "B"(w117) -> ()
            n608 = local write "C"(w117) -> ()
          }
          frame 336..419 {
            w119 = FALSE
            n609 = local write "E"(TRUE) -> ()
            n610 = local write "F"(w119) -> ()
            n611 = local write "F#"(w119) -> ()
            n612 = local write "G"(w119) -> ()
            n613 = local write "G#"(w119) -> ()
            n614 = local write "STANDBY"(w119) -> ()
            n615 = local write "C#"(w119) -> ()
            n616 = local write "D"(w119) -> ()
            n617 = local write "D#"(w119) -> ()
            n618 = local write "A"(w119) -> ()
            n619 = local write "A#"(w119) -> ()
            n620 = local write "B"(w119) -> ()
            n621 = local write "C"(w119) -> ()
          }
          frame 420..503 {
            w121 = FALSE
            n622 = local write "F"(TRUE) -> ()
            n623 = local write "STANDBY"(w121) -> ()
            n624 = local write "F#"(w121) -> ()
            n625 = local write "G"(w121) -> ()
            n626 = local write "G#"(w121) -> ()
            n627 = local write "C#"(w121) -> ()
            n628 = local write "D"(w121) -> ()
            n629 = local write "D#"(w121) -> ()
            n630 = local write "E"(w121) -> ()
            n631 = local write "A"(w121) -> ()
            n632 = local write "A#"(w121) -> ()
            n633 = local write "B"(w121) -> ()
            n634 = local write "C"(w121) -> ()
          }
          frame 504..587 {
            w123 = FALSE
            n635 = local write "F#"(TRUE) -> ()
            n636 = local write "STANDBY"(w123) -> ()
            n637 = local write "F"(w123) -> ()
            n638 = local write "G"(w123) -> ()
            n639 = local write "G#"(w123) -> ()
            n640 = local write "C#"(w123) -> ()
            n641 = local write "D"(w123) -> ()
            n642 = local write "D#"(w123) -> ()
            n643 = local write "E"(w123) -> ()
            n644 = local write "A"(w123) -> ()
            n645 = local write "A#"(w123) -> ()
            n646 = local write "B"(w123) -> ()
            n647 = local write "C"(w123) -> ()
          }
          frame 588..671 {
            w125 = FALSE
            n648 = local write "G"(TRUE) -> ()
            n649 = local write "STANDBY"(w125) -> ()
            n650 = local write "F"(w125) -> ()
            n651 = local write "F#"(w125) -> ()
            n652 = local write "G#"(w125) -> ()
            n653 = local write "C#"(w125) -> ()
            n654 = local write "D"(w125) -> ()
            n655 = local write "D#"(w125) -> ()
            n656 = local write "E"(w125) -> ()
            n657 = local write "A"(w125) -> ()
            n658 = local write "A#"(w125) -> ()
            n659 = local write "B"(w125) -> ()
            n660 = local write "C"(w125) -> ()
          }
          frame 672..755 {
            w127 = FALSE
            n661 = local write "G#"(TRUE) -> ()
            n662 = local write "STANDBY"(w127) -> ()
            n663 = local write "F"(w127) -> ()
            n664 = local write "F#"(w127) -> ()
            n665 = local write "G"(w127) -> ()
            n666 = local write "C#"(w127) -> ()
            n667 = local write "D"(w127) -> ()
            n668 = local write "D#"(w127) -> ()
            n669 = local write "E"(w127) -> ()
            n670 = local write "A"(w127) -> ()
            n671 = local write "A#"(w127) -> ()
            n672 = local write "B"(w127) -> ()
            n673 = local write "C"(w127) -> ()
          }
          frame 756..839 {
            w129 = FALSE
            n674 = local write "A"(TRUE) -> ()
            n675 = local write "F"(w129) -> ()
            n676 = local write "F#"(w129) -> ()
            n677 = local write "G"(w129) -> ()
            n678 = local write "G#"(w129) -> ()
            n679 = local write "C#"(w129) -> ()
            n680 = local write "D"(w129) -> ()
            n681 = local write "D#"(w129) -> ()
            n682 = local write "E"(w129) -> ()
            n683 = local write "STANDBY"(w129) -> ()
            n684 = local write "A#"(w129) -> ()
            n685 = local write "B"(w129) -> ()
            n686 = local write "C"(w129) -> ()
          }
          frame 840..923 {
            w131 = FALSE
            n687 = local write "A#"(TRUE) -> ()
            n688 = local write "F"(w131) -> ()
            n689 = local write "F#"(w131) -> ()
            n690 = local write "G"(w131) -> ()
            n691 = local write "G#"(w131) -> ()
            n692 = local write "C#"(w131) -> ()
            n693 = local write "D"(w131) -> ()
            n694 = local write "D#"(w131) -> ()
            n695 = local write "E"(w131) -> ()
            n696 = local write "STANDBY"(w131) -> ()
            n697 = local write "A"(w131) -> ()
            n698 = local write "B"(w131) -> ()
            n699 = local write "C"(w131) -> ()
          }
          frame 924..1000 {
            w133 = FALSE
            n700 = local write "B"(TRUE) -> ()
            n701 = local write "F"(w133) -> ()
            n702 = local write "F#"(w133) -> ()
            n703 = local write "G"(w133) -> ()
            n704 = local write "G#"(w133) -> ()
            n705 = local write "C#"(w133) -> ()
            n706 = local write "D"(w133) -> ()
            n707 = local write "D#"(w133) -> ()
            n708 = local write "E"(w133) -> ()
            n709 = local write "STANDBY"(w133) -> ()
            n710 = local write "A"(w133) -> ()
            n711 = local write "A#"(w133) -> ()
            n712 = local write "C"(w133) -> ()
          }
        }
        n713 = local write "Octave 3"(TRUE) -> ()
        n714 = local write "Octave 4"(w106) -> ()
        n715 = local write "Octave 2"(w106) -> ()
        n716 = local write "Octave 1"(w106) -> ()
        n717 = local write "Octave 0"(w106) -> ()
        n718 = local write "Octave 5"(w106) -> ()
        n719 = local write "Octave 8"(w106) -> ()
        n720 = local write "Octave 7"(w106) -> ()
        n721 = local write "Octave 6"(w106) -> ()
      }
      frame 113..140 {
        w135 = FALSE
        n722 = case shown="0, Default" w137 {
          frame 0, Default {
            w138 = FALSE
            n723 = local write "STANDBY"(TRUE) -> ()
            n724 = local write "F"(w138) -> ()
            n725 = local write "F#"(w138) -> ()
            n726 = local write "G"(w138) -> ()
            n727 = local write "G#"(w138) -> ()
            n728 = local write "C#"(w138) -> ()
            n729 = local write "D"(w138) -> ()
            n730 = local write "D#"(w138) -> ()
            n731 = local write "E"(w138) -> ()
            n732 = local write "A"(w138) -> ()
            n733 = local write "A#"(w138) -> ()
            n734 = local write "B"(w138) -> ()
            n735 = local write "C"(w138) -> ()
          }
          frame 1..83 {
            w140 = FALSE
            n736 = local write "C"(TRUE) -> ()
            n737 = local write "F"(w140) -> ()
            n738 = local write "F#"(w140) -> ()
            n739 = local write "G"(w140) -> ()
            n740 = local write "G#"(w140) -> ()
            n741 = local write "C#"(w140) -> ()
            n742 = local write "D"(w140) -> ()
            n743 = local write "D#"(w140) -> ()
            n744 = local write "E"(w140) -> ()
            n745 = local write "STANDBY"(w140) -> ()
            n746 = local write "A"(w140) -> ()
            n747 = local write "A#"(w140) -> ()
            n748 = local write "B"(w140) -> ()
          }
          frame 84..167 {
            w142 = FALSE
            n749 = local write "C#"(TRUE) -> ()
            n750 = local write "F"(w142) -> ()
            n751 = local write "F#"(w142) -> ()
            n752 = local write "G"(w142) -> ()
            n753 = local write "G#"(w142) -> ()
            n754 = local write "STANDBY"(w142) -> ()
            n755 = local write "D"(w142) -> ()
            n756 = local write "D#"(w142) -> ()
            n757 = local write "E"(w142) -> ()
            n758 = local write "A"(w142) -> ()
            n759 = local write "A#"(w142) -> ()
            n760 = local write "B"(w142) -> ()
            n761 = local write "C"(w142) -> ()
          }
          frame 168..251 {
            w144 = FALSE
            n762 = local write "D"(TRUE) -> ()
            n763 = local write "F"(w144) -> ()
            n764 = local write "F#"(w144) -> ()
            n765 = local write "G"(w144) -> ()
            n766 = local write "G#"(w144) -> ()
            n767 = local write "STANDBY"(w144) -> ()
            n768 = local write "C#"(w144) -> ()
            n769 = local write "D#"(w144) -> ()
            n770 = local write "E"(w144) -> ()
            n771 = local write "A"(w144) -> ()
            n772 = local write "A#"(w144) -> ()
            n773 = local write "B"(w144) -> ()
            n774 = local write "C"(w144) -> ()
          }
          frame 252..335 {
            w146 = FALSE
            n775 = local write "D#"(TRUE) -> ()
            n776 = local write "F"(w146) -> ()
            n777 = local write "F#"(w146) -> ()
            n778 = local write "G"(w146) -> ()
            n779 = local write "G#"(w146) -> ()
            n780 = local write "STANDBY"(w146) -> ()
            n781 = local write "C#"(w146) -> ()
            n782 = local write "D"(w146) -> ()
            n783 = local write "E"(w146) -> ()
            n784 = local write "A"(w146) -> ()
            n785 = local write "A#"(w146) -> ()
            n786 = local write "B"(w146) -> ()
            n787 = local write "C"(w146) -> ()
          }
          frame 336..419 {
            w148 = FALSE
            n788 = local write "E"(TRUE) -> ()
            n789 = local write "F"(w148) -> ()
            n790 = local write "F#"(w148) -> ()
            n791 = local write "G"(w148) -> ()
            n792 = local write "G#"(w148) -> ()
            n793 = local write "STANDBY"(w148) -> ()
            n794 = local write "C#"(w148) -> ()
            n795 = local write "D"(w148) -> ()
            n796 = local write "D#"(w148) -> ()
            n797 = local write "A"(w148) -> ()
            n798 = local write "A#"(w148) -> ()
            n799 = local write "B"(w148) -> ()
            n800 = local write "C"(w148) -> ()
          }
          frame 420..503 {
            w150 = FALSE
            n801 = local write "F"(TRUE) -> ()
            n802 = local write "STANDBY"(w150) -> ()
            n803 = local write "F#"(w150) -> ()
            n804 = local write "G"(w150) -> ()
            n805 = local write "G#"(w150) -> ()
            n806 = local write "C#"(w150) -> ()
            n807 = local write "D"(w150) -> ()
            n808 = local write "D#"(w150) -> ()
            n809 = local write "E"(w150) -> ()
            n810 = local write "A"(w150) -> ()
            n811 = local write "A#"(w150) -> ()
            n812 = local write "B"(w150) -> ()
            n813 = local write "C"(w150) -> ()
          }
          frame 504..587 {
            w152 = FALSE
            n814 = local write "F#"(TRUE) -> ()
            n815 = local write "STANDBY"(w152) -> ()
            n816 = local write "F"(w152) -> ()
            n817 = local write "G"(w152) -> ()
            n818 = local write "G#"(w152) -> ()
            n819 = local write "C#"(w152) -> ()
            n820 = local write "D"(w152) -> ()
            n821 = local write "D#"(w152) -> ()
            n822 = local write "E"(w152) -> ()
            n823 = local write "A"(w152) -> ()
            n824 = local write "A#"(w152) -> ()
            n825 = local write "B"(w152) -> ()
            n826 = local write "C"(w152) -> ()
          }
          frame 588..671 {
            w154 = FALSE
            n827 = local write "G"(TRUE) -> ()
            n828 = local write "STANDBY"(w154) -> ()
            n829 = local write "F"(w154) -> ()
            n830 = local write "F#"(w154) -> ()
            n831 = local write "G#"(w154) -> ()
            n832 = local write "C#"(w154) -> ()
            n833 = local write "D"(w154) -> ()
            n834 = local write "D#"(w154) -> ()
            n835 = local write "E"(w154) -> ()
            n836 = local write "A"(w154) -> ()
            n837 = local write "A#"(w154) -> ()
            n838 = local write "B"(w154) -> ()
            n839 = local write "C"(w154) -> ()
          }
          frame 672..755 {
            w156 = FALSE
            n840 = local write "G#"(TRUE) -> ()
            n841 = local write "STANDBY"(w156) -> ()
            n842 = local write "F"(w156) -> ()
            n843 = local write "F#"(w156) -> ()
            n844 = local write "G"(w156) -> ()
            n845 = local write "C#"(w156) -> ()
            n846 = local write "D"(w156) -> ()
            n847 = local write "D#"(w156) -> ()
            n848 = local write "E"(w156) -> ()
            n849 = local write "A"(w156) -> ()
            n850 = local write "A#"(w156) -> ()
            n851 = local write "B"(w156) -> ()
            n852 = local write "C"(w156) -> ()
          }
          frame 756..839 {
            w158 = FALSE
            n853 = local write "A"(TRUE) -> ()
            n854 = local write "F"(w158) -> ()
            n855 = local write "F#"(w158) -> ()
            n856 = local write "G"(w158) -> ()
            n857 = local write "G#"(w158) -> ()
            n858 = local write "C#"(w158) -> ()
            n859 = local write "D"(w158) -> ()
            n860 = local write "D#"(w158) -> ()
            n861 = local write "E"(w158) -> ()
            n862 = local write "STANDBY"(w158) -> ()
            n863 = local write "A#"(w158) -> ()
            n864 = local write "B"(w158) -> ()
            n865 = local write "C"(w158) -> ()
          }
          frame 840..923 {
            w160 = FALSE
            n866 = local write "A#"(TRUE) -> ()
            n867 = local write "F"(w160) -> ()
            n868 = local write "F#"(w160) -> ()
            n869 = local write "G"(w160) -> ()
            n870 = local write "G#"(w160) -> ()
            n871 = local write "C#"(w160) -> ()
            n872 = local write "D"(w160) -> ()
            n873 = local write "D#"(w160) -> ()
            n874 = local write "E"(w160) -> ()
            n875 = local write "STANDBY"(w160) -> ()
            n876 = local write "A"(w160) -> ()
            n877 = local write "B"(w160) -> ()
            n878 = local write "C"(w160) -> ()
          }
          frame 924..1000 {
            w162 = FALSE
            n879 = local write "B"(TRUE) -> ()
            n880 = local write "F"(w162) -> ()
            n881 = local write "F#"(w162) -> ()
            n882 = local write "G"(w162) -> ()
            n883 = local write "G#"(w162) -> ()
            n884 = local write "C#"(w162) -> ()
            n885 = local write "D"(w162) -> ()
            n886 = local write "D#"(w162) -> ()
            n887 = local write "E"(w162) -> ()
            n888 = local write "STANDBY"(w162) -> ()
            n889 = local write "A"(w162) -> ()
            n890 = local write "A#"(w162) -> ()
            n891 = local write "C"(w162) -> ()
          }
        }
        n892 = local write "Octave 4"(TRUE) -> ()
        n893 = local write "Octave 3"(w135) -> ()
        n894 = local write "Octave 2"(w135) -> ()
        n895 = local write "Octave 1"(w135) -> ()
        n896 = local write "Octave 0"(w135) -> ()
        n897 = local write "Octave 5"(w135) -> ()
        n898 = local write "Octave 8"(w135) -> ()
        n899 = local write "Octave 7"(w135) -> ()
        n900 = local write "Octave 6"(w135) -> ()
      }
      frame 141..168 {
        w164 = FALSE
        n901 = case shown="0, Default" w166 {
          frame 0, Default {
            w167 = FALSE
            n902 = local write "STANDBY"(TRUE) -> ()
            n903 = local write "F"(w167) -> ()
            n904 = local write "F#"(w167) -> ()
            n905 = local write "G"(w167) -> ()
            n906 = local write "G#"(w167) -> ()
            n907 = local write "C#"(w167) -> ()
            n908 = local write "D"(w167) -> ()
            n909 = local write "D#"(w167) -> ()
            n910 = local write "E"(w167) -> ()
            n911 = local write "A"(w167) -> ()
            n912 = local write "A#"(w167) -> ()
            n913 = local write "B"(w167) -> ()
            n914 = local write "C"(w167) -> ()
          }
          frame 1..83 {
            w169 = FALSE
            n915 = local write "C"(TRUE) -> ()
            n916 = local write "F"(w169) -> ()
            n917 = local write "F#"(w169) -> ()
            n918 = local write "G"(w169) -> ()
            n919 = local write "G#"(w169) -> ()
            n920 = local write "C#"(w169) -> ()
            n921 = local write "D"(w169) -> ()
            n922 = local write "D#"(w169) -> ()
            n923 = local write "E"(w169) -> ()
            n924 = local write "STANDBY"(w169) -> ()
            n925 = local write "A"(w169) -> ()
            n926 = local write "A#"(w169) -> ()
            n927 = local write "B"(w169) -> ()
          }
          frame 84..167 {
            w171 = FALSE
            n928 = local write "C#"(TRUE) -> ()
            n929 = local write "F"(w171) -> ()
            n930 = local write "F#"(w171) -> ()
            n931 = local write "G"(w171) -> ()
            n932 = local write "G#"(w171) -> ()
            n933 = local write "STANDBY"(w171) -> ()
            n934 = local write "D"(w171) -> ()
            n935 = local write "D#"(w171) -> ()
            n936 = local write "E"(w171) -> ()
            n937 = local write "A"(w171) -> ()
            n938 = local write "A#"(w171) -> ()
            n939 = local write "B"(w171) -> ()
            n940 = local write "C"(w171) -> ()
          }
          frame 168..251 {
            w173 = FALSE
            n941 = local write "D"(TRUE) -> ()
            n942 = local write "F"(w173) -> ()
            n943 = local write "F#"(w173) -> ()
            n944 = local write "G"(w173) -> ()
            n945 = local write "G#"(w173) -> ()
            n946 = local write "STANDBY"(w173) -> ()
            n947 = local write "C#"(w173) -> ()
            n948 = local write "D#"(w173) -> ()
            n949 = local write "E"(w173) -> ()
            n950 = local write "A"(w173) -> ()
            n951 = local write "A#"(w173) -> ()
            n952 = local write "B"(w173) -> ()
            n953 = local write "C"(w173) -> ()
          }
          frame 252..335 {
            w175 = FALSE
            n954 = local write "D#"(TRUE) -> ()
            n955 = local write "F"(w175) -> ()
            n956 = local write "F#"(w175) -> ()
            n957 = local write "G"(w175) -> ()
            n958 = local write "G#"(w175) -> ()
            n959 = local write "STANDBY"(w175) -> ()
            n960 = local write "C#"(w175) -> ()
            n961 = local write "D"(w175) -> ()
            n962 = local write "E"(w175) -> ()
            n963 = local write "A"(w175) -> ()
            n964 = local write "A#"(w175) -> ()
            n965 = local write "B"(w175) -> ()
            n966 = local write "C"(w175) -> ()
          }
          frame 336..419 {
            w177 = FALSE
            n967 = local write "E"(TRUE) -> ()
            n968 = local write "F"(w177) -> ()
            n969 = local write "F#"(w177) -> ()
            n970 = local write "G"(w177) -> ()
            n971 = local write "G#"(w177) -> ()
            n972 = local write "STANDBY"(w177) -> ()
            n973 = local write "C#"(w177) -> ()
            n974 = local write "D"(w177) -> ()
            n975 = local write "D#"(w177) -> ()
            n976 = local write "A"(w177) -> ()
            n977 = local write "A#"(w177) -> ()
            n978 = local write "B"(w177) -> ()
            n979 = local write "C"(w177) -> ()
          }
          frame 420..503 {
            w179 = FALSE
            n980 = local write "F"(TRUE) -> ()
            n981 = local write "STANDBY"(w179) -> ()
            n982 = local write "F#"(w179) -> ()
            n983 = local write "G"(w179) -> ()
            n984 = local write "G#"(w179) -> ()
            n985 = local write "C#"(w179) -> ()
            n986 = local write "D"(w179) -> ()
            n987 = local write "D#"(w179) -> ()
            n988 = local write "E"(w179) -> ()
            n989 = local write "A"(w179) -> ()
            n990 = local write "A#"(w179) -> ()
            n991 = local write "B"(w179) -> ()
            n992 = local write "C"(w179) -> ()
          }
          frame 504..587 {
            w181 = FALSE
            n993 = local write "F#"(TRUE) -> ()
            n994 = local write "STANDBY"(w181) -> ()
            n995 = local write "F"(w181) -> ()
            n996 = local write "G"(w181) -> ()
            n997 = local write "G#"(w181) -> ()
            n998 = local write "C#"(w181) -> ()
            n999 = local write "D"(w181) -> ()
            n1000 = local write "D#"(w181) -> ()
            n1001 = local write "E"(w181) -> ()
            n1002 = local write "A"(w181) -> ()
            n1003 = local write "A#"(w181) -> ()
            n1004 = local write "B"(w181) -> ()
            n1005 = local write "C"(w181) -> ()
          }
          frame 588..671 {
            w183 = FALSE
            n1006 = local write "G"(TRUE) -> ()
            n1007 = local write "STANDBY"(w183) -> ()
            n1008 = local write "F"(w183) -> ()
            n1009 = local write "F#"(w183) -> ()
            n1010 = local write "G#"(w183) -> ()
            n1011 = local write "C#"(w183) -> ()
            n1012 = local write "D"(w183) -> ()
            n1013 = local write "D#"(w183) -> ()
            n1014 = local write "E"(w183) -> ()
            n1015 = local write "A"(w183) -> ()
            n1016 = local write "A#"(w183) -> ()
            n1017 = local write "B"(w183) -> ()
            n1018 = local write "C"(w183) -> ()
          }
          frame 672..755 {
            w185 = FALSE
            n1019 = local write "G#"(TRUE) -> ()
            n1020 = local write "STANDBY"(w185) -> ()
            n1021 = local write "F"(w185) -> ()
            n1022 = local write "F#"(w185) -> ()
            n1023 = local write "G"(w185) -> ()
            n1024 = local write "C#"(w185) -> ()
            n1025 = local write "D"(w185) -> ()
            n1026 = local write "D#"(w185) -> ()
            n1027 = local write "E"(w185) -> ()
            n1028 = local write "A"(w185) -> ()
            n1029 = local write "A#"(w185) -> ()
            n1030 = local write "B"(w185) -> ()
            n1031 = local write "C"(w185) -> ()
          }
          frame 756..839 {
            w187 = FALSE
            n1032 = local write "A"(TRUE) -> ()
            n1033 = local write "F"(w187) -> ()
            n1034 = local write "F#"(w187) -> ()
            n1035 = local write "G"(w187) -> ()
            n1036 = local write "G#"(w187) -> ()
            n1037 = local write "C#"(w187) -> ()
            n1038 = local write "D"(w187) -> ()
            n1039 = local write "D#"(w187) -> ()
            n1040 = local write "E"(w187) -> ()
            n1041 = local write "STANDBY"(w187) -> ()
            n1042 = local write "A#"(w187) -> ()
            n1043 = local write "B"(w187) -> ()
            n1044 = local write "C"(w187) -> ()
          }
          frame 840..923 {
            w189 = FALSE
            n1045 = local write "A#"(TRUE) -> ()
            n1046 = local write "F"(w189) -> ()
            n1047 = local write "F#"(w189) -> ()
            n1048 = local write "G"(w189) -> ()
            n1049 = local write "G#"(w189) -> ()
            n1050 = local write "C#"(w189) -> ()
            n1051 = local write "D"(w189) -> ()
            n1052 = local write "D#"(w189) -> ()
            n1053 = local write "E"(w189) -> ()
            n1054 = local write "STANDBY"(w189) -> ()
            n1055 = local write "A"(w189) -> ()
            n1056 = local write "B"(w189) -> ()
            n1057 = local write "C"(w189) -> ()
          }
          frame 924..1000 {
            w191 = FALSE
            n1058 = local write "B"(TRUE) -> ()
            n1059 = local write "F"(w191) -> ()
            n1060 = local write "F#"(w191) -> ()
            n1061 = local write "G"(w191) -> ()
            n1062 = local write "G#"(w191) -> ()
            n1063 = local write "C#"(w191) -> ()
            n1064 = local write "D"(w191) -> ()
            n1065 = local write "D#"(w191) -> ()
            n1066 = local write "E"(w191) -> ()
            n1067 = local write "STANDBY"(w191) -> ()
            n1068 = local write "A"(w191) -> ()
            n1069 = local write "A#"(w191) -> ()
            n1070 = local write "C"(w191) -> ()
          }
        }
        n1071 = local write "Octave 5"(TRUE) -> ()
        n1072 = local write "Octave 3"(w164) -> ()
        n1073 = local write "Octave 2"(w164) -> ()
        n1074 = local write "Octave 1"(w164) -> ()
        n1075 = local write "Octave 0"(w164) -> ()
        n1076 = local write "Octave 4"(w164) -> ()
        n1077 = local write "Octave 8"(w164) -> ()
        n1078 = local write "Octave 7"(w164) -> ()
        n1079 = local write "Octave 6"(w164) -> ()
      }
      frame 169..196 {
        w193 = FALSE
        n1080 = case shown="924.." w195 {
          frame 0, Default {
            w196 = FALSE
            n1081 = local write "STANDBY"(TRUE) -> ()
            n1082 = local write "F"(w196) -> ()
            n1083 = local write "F#"(w196) -> ()
            n1084 = local write "G"(w196) -> ()
            n1085 = local write "G#"(w196) -> ()
            n1086 = local write "C#"(w196) -> ()
            n1087 = local write "D"(w196) -> ()
            n1088 = local write "D#"(w196) -> ()
            n1089 = local write "E"(w196) -> ()
            n1090 = local write "A"(w196) -> ()
            n1091 = local write "A#"(w196) -> ()
            n1092 = local write "B"(w196) -> ()
            n1093 = local write "C"(w196) -> ()
          }
          frame 1..83 {
            w198 = FALSE
            n1094 = local write "C"(TRUE) -> ()
            n1095 = local write "F"(w198) -> ()
            n1096 = local write "F#"(w198) -> ()
            n1097 = local write "G"(w198) -> ()
            n1098 = local write "G#"(w198) -> ()
            n1099 = local write "C#"(w198) -> ()
            n1100 = local write "D"(w198) -> ()
            n1101 = local write "D#"(w198) -> ()
            n1102 = local write "E"(w198) -> ()
            n1103 = local write "STANDBY"(w198) -> ()
            n1104 = local write "A"(w198) -> ()
            n1105 = local write "A#"(w198) -> ()
            n1106 = local write "B"(w198) -> ()
          }
          frame 84..167 {
            w200 = FALSE
            n1107 = local write "C#"(TRUE) -> ()
            n1108 = local write "F"(w200) -> ()
            n1109 = local write "F#"(w200) -> ()
            n1110 = local write "G"(w200) -> ()
            n1111 = local write "G#"(w200) -> ()
            n1112 = local write "STANDBY"(w200) -> ()
            n1113 = local write "D"(w200) -> ()
            n1114 = local write "D#"(w200) -> ()
            n1115 = local write "E"(w200) -> ()
            n1116 = local write "A"(w200) -> ()
            n1117 = local write "A#"(w200) -> ()
            n1118 = local write "B"(w200) -> ()
            n1119 = local write "C"(w200) -> ()
          }
          frame 168..251 {
            w202 = FALSE
            n1120 = local write "D"(TRUE) -> ()
            n1121 = local write "F"(w202) -> ()
            n1122 = local write "F#"(w202) -> ()
            n1123 = local write "G"(w202) -> ()
            n1124 = local write "G#"(w202) -> ()
            n1125 = local write "STANDBY"(w202) -> ()
            n1126 = local write "C#"(w202) -> ()
            n1127 = local write "D#"(w202) -> ()
            n1128 = local write "E"(w202) -> ()
            n1129 = local write "A"(w202) -> ()
            n1130 = local write "A#"(w202) -> ()
            n1131 = local write "B"(w202) -> ()
            n1132 = local write "C"(w202) -> ()
          }
          frame 252..335 {
            w204 = FALSE
            n1133 = local write "D#"(TRUE) -> ()
            n1134 = local write "F"(w204) -> ()
            n1135 = local write "F#"(w204) -> ()
            n1136 = local write "G"(w204) -> ()
            n1137 = local write "G#"(w204) -> ()
            n1138 = local write "STANDBY"(w204) -> ()
            n1139 = local write "C#"(w204) -> ()
            n1140 = local write "D"(w204) -> ()
            n1141 = local write "E"(w204) -> ()
            n1142 = local write "A"(w204) -> ()
            n1143 = local write "A#"(w204) -> ()
            n1144 = local write "B"(w204) -> ()
            n1145 = local write "C"(w204) -> ()
          }
          frame 336..419 {
            w206 = FALSE
            n1146 = local write "E"(TRUE) -> ()
            n1147 = local write "F"(w206) -> ()
            n1148 = local write "F#"(w206) -> ()
            n1149 = local write "G"(w206) -> ()
            n1150 = local write "G#"(w206) -> ()
            n1151 = local write "STANDBY"(w206) -> ()
            n1152 = local write "C#"(w206) -> ()
            n1153 = local write "D"(w206) -> ()
            n1154 = local write "D#"(w206) -> ()
            n1155 = local write "A"(w206) -> ()
            n1156 = local write "A#"(w206) -> ()
            n1157 = local write "B"(w206) -> ()
            n1158 = local write "C"(w206) -> ()
          }
          frame 420..503 {
            w208 = FALSE
            n1159 = local write "F"(TRUE) -> ()
            n1160 = local write "STANDBY"(w208) -> ()
            n1161 = local write "F#"(w208) -> ()
            n1162 = local write "G"(w208) -> ()
            n1163 = local write "G#"(w208) -> ()
            n1164 = local write "C#"(w208) -> ()
            n1165 = local write "D"(w208) -> ()
            n1166 = local write "D#"(w208) -> ()
            n1167 = local write "E"(w208) -> ()
            n1168 = local write "A"(w208) -> ()
            n1169 = local write "A#"(w208) -> ()
            n1170 = local write "B"(w208) -> ()
            n1171 = local write "C"(w208) -> ()
          }
          frame 504..587 {
            w210 = FALSE
            n1172 = local write "F#"(TRUE) -> ()
            n1173 = local write "STANDBY"(w210) -> ()
            n1174 = local write "F"(w210) -> ()
            n1175 = local write "G"(w210) -> ()
            n1176 = local write "G#"(w210) -> ()
            n1177 = local write "C#"(w210) -> ()
            n1178 = local write "D"(w210) -> ()
            n1179 = local write "D#"(w210) -> ()
            n1180 = local write "E"(w210) -> ()
            n1181 = local write "A"(w210) -> ()
            n1182 = local write "A#"(w210) -> ()
            n1183 = local write "B"(w210) -> ()
            n1184 = local write "C"(w210) -> ()
          }
          frame 588..671 {
            w212 = FALSE
            n1185 = local write "G"(TRUE) -> ()
            n1186 = local write "STANDBY"(w212) -> ()
            n1187 = local write "F"(w212) -> ()
            n1188 = local write "F#"(w212) -> ()
            n1189 = local write "G#"(w212) -> ()
            n1190 = local write "C#"(w212) -> ()
            n1191 = local write "D"(w212) -> ()
            n1192 = local write "D#"(w212) -> ()
            n1193 = local write "E"(w212) -> ()
            n1194 = local write "A"(w212) -> ()
            n1195 = local write "A#"(w212) -> ()
            n1196 = local write "B"(w212) -> ()
            n1197 = local write "C"(w212) -> ()
          }
          frame 672..755 {
            w214 = FALSE
            n1198 = local write "G#"(TRUE) -> ()
            n1199 = local write "STANDBY"(w214) -> ()
            n1200 = local write "F"(w214) -> ()
            n1201 = local write "F#"(w214) -> ()
            n1202 = local write "G"(w214) -> ()
            n1203 = local write "C#"(w214) -> ()
            n1204 = local write "D"(w214) -> ()
            n1205 = local write "D#"(w214) -> ()
            n1206 = local write "E"(w214) -> ()
            n1207 = local write "A"(w214) -> ()
            n1208 = local write "A#"(w214) -> ()
            n1209 = local write "B"(w214) -> ()
            n1210 = local write "C"(w214) -> ()
          }
          frame 756..839 {
            w216 = FALSE
            n1211 = local write "A"(TRUE) -> ()
            n1212 = local write "F"(w216) -> ()
            n1213 = local write "F#"(w216) -> ()
            n1214 = local write "G"(w216) -> ()
            n1215 = local write "G#"(w216) -> ()
            n1216 = local write "C#"(w216) -> ()
            n1217 = local write "D"(w216) -> ()
            n1218 = local write "D#"(w216) -> ()
            n1219 = local write "E"(w216) -> ()
            n1220 = local write "STANDBY"(w216) -> ()
            n1221 = local write "A#"(w216) -> ()
            n1222 = local write "B"(w216) -> ()
            n1223 = local write "C"(w216) -> ()
          }
          frame 840..923 {
            w218 = FALSE
            n1224 = local write "A#"(TRUE) -> ()
            n1225 = local write "F"(w218) -> ()
            n1226 = local write "F#"(w218) -> ()
            n1227 = local write "G"(w218) -> ()
            n1228 = local write "G#"(w218) -> ()
            n1229 = local write "C#"(w218) -> ()
            n1230 = local write "D"(w218) -> ()
            n1231 = local write "D#"(w218) -> ()
            n1232 = local write "E"(w218) -> ()
            n1233 = local write "STANDBY"(w218) -> ()
            n1234 = local write "A"(w218) -> ()
            n1235 = local write "B"(w218) -> ()
            n1236 = local write "C"(w218) -> ()
          }
          frame 924.. {
            w220 = FALSE
            n1237 = local write "B"(TRUE) -> ()
            n1238 = local write "F"(w220) -> ()
            n1239 = local write "F#"(w220) -> ()
            n1240 = local write "G"(w220) -> ()
            n1241 = local write "G#"(w220) -> ()
            n1242 = local write "C#"(w220) -> ()
            n1243 = local write "D"(w220) -> ()
            n1244 = local write "D#"(w220) -> ()
            n1245 = local write "E"(w220) -> ()
            n1246 = local write "STANDBY"(w220) -> ()
            n1247 = local write "A"(w220) -> ()
            n1248 = local write "A#"(w220) -> ()
            n1249 = local write "C"(w220) -> ()
          }
        }
        n1250 = local write "Octave 6"(TRUE) -> ()
        n1251 = local write "Octave 3"(w193) -> ()
        n1252 = local write "Octave 2"(w193) -> ()
        n1253 = local write "Octave 1"(w193) -> ()
        n1254 = local write "Octave 0"(w193) -> ()
        n1255 = local write "Octave 4"(w193) -> ()
        n1256 = local write "Octave 8"(w193) -> ()
        n1257 = local write "Octave 7"(w193) -> ()
        n1258 = local write "Octave 5"(w193) -> ()
      }
      frame 197..224 {
        w222 = FALSE
        n1259 = case shown="0, Default" w224 {
          frame 0, Default {
            w225 = FALSE
            n1260 = local write "STANDBY"(TRUE) -> ()
            n1261 = local write "F"(w225) -> ()
            n1262 = local write "F#"(w225) -> ()
            n1263 = local write "G"(w225) -> ()
            n1264 = local write "G#"(w225) -> ()
            n1265 = local write "C#"(w225) -> ()
            n1266 = local write "D"(w225) -> ()
            n1267 = local write "D#"(w225) -> ()
            n1268 = local write "E"(w225) -> ()
            n1269 = local write "A"(w225) -> ()
            n1270 = local write "A#"(w225) -> ()
            n1271 = local write "B"(w225) -> ()
            n1272 = local write "C"(w225) -> ()
          }
          frame 1..83 {
            w227 = FALSE
            n1273 = local write "C"(TRUE) -> ()
            n1274 = local write "F"(w227) -> ()
            n1275 = local write "F#"(w227) -> ()
            n1276 = local write "G"(w227) -> ()
            n1277 = local write "G#"(w227) -> ()
            n1278 = local write "C#"(w227) -> ()
            n1279 = local write "D"(w227) -> ()
            n1280 = local write "D#"(w227) -> ()
            n1281 = local write "E"(w227) -> ()
            n1282 = local write "STANDBY"(w227) -> ()
            n1283 = local write "A"(w227) -> ()
            n1284 = local write "A#"(w227) -> ()
            n1285 = local write "B"(w227) -> ()
          }
          frame 84..167 {
            w229 = FALSE
            n1286 = local write "C#"(TRUE) -> ()
            n1287 = local write "F"(w229) -> ()
            n1288 = local write "F#"(w229) -> ()
            n1289 = local write "G"(w229) -> ()
            n1290 = local write "G#"(w229) -> ()
            n1291 = local write "STANDBY"(w229) -> ()
            n1292 = local write "D"(w229) -> ()
            n1293 = local write "D#"(w229) -> ()
            n1294 = local write "E"(w229) -> ()
            n1295 = local write "A"(w229) -> ()
            n1296 = local write "A#"(w229) -> ()
            n1297 = local write "B"(w229) -> ()
            n1298 = local write "C"(w229) -> ()
          }
          frame 168..251 {
            w231 = FALSE
            n1299 = local write "D"(TRUE) -> ()
            n1300 = local write "F"(w231) -> ()
            n1301 = local write "F#"(w231) -> ()
            n1302 = local write "G"(w231) -> ()
            n1303 = local write "G#"(w231) -> ()
            n1304 = local write "STANDBY"(w231) -> ()
            n1305 = local write "C#"(w231) -> ()
            n1306 = local write "D#"(w231) -> ()
            n1307 = local write "E"(w231) -> ()
            n1308 = local write "A"(w231) -> ()
            n1309 = local write "A#"(w231) -> ()
            n1310 = local write "B"(w231) -> ()
            n1311 = local write "C"(w231) -> ()
          }
          frame 252..335 {
            w233 = FALSE
            n1312 = local write "D#"(TRUE) -> ()
            n1313 = local write "F"(w233) -> ()
            n1314 = local write "F#"(w233) -> ()
            n1315 = local write "G"(w233) -> ()
            n1316 = local write "G#"(w233) -> ()
            n1317 = local write "STANDBY"(w233) -> ()
            n1318 = local write "C#"(w233) -> ()
            n1319 = local write "D"(w233) -> ()
            n1320 = local write "E"(w233) -> ()
            n1321 = local write "A"(w233) -> ()
            n1322 = local write "A#"(w233) -> ()
            n1323 = local write "B"(w233) -> ()
            n1324 = local write "C"(w233) -> ()
          }
          frame 336..419 {
            w235 = FALSE
            n1325 = local write "E"(TRUE) -> ()
            n1326 = local write "F"(w235) -> ()
            n1327 = local write "F#"(w235) -> ()
            n1328 = local write "G"(w235) -> ()
            n1329 = local write "G#"(w235) -> ()
            n1330 = local write "STANDBY"(w235) -> ()
            n1331 = local write "C#"(w235) -> ()
            n1332 = local write "D"(w235) -> ()
            n1333 = local write "D#"(w235) -> ()
            n1334 = local write "A"(w235) -> ()
            n1335 = local write "A#"(w235) -> ()
            n1336 = local write "B"(w235) -> ()
            n1337 = local write "C"(w235) -> ()
          }
          frame 420..503 {
            w237 = FALSE
            n1338 = local write "F"(TRUE) -> ()
            n1339 = local write "STANDBY"(w237) -> ()
            n1340 = local write "F#"(w237) -> ()
            n1341 = local write "G"(w237) -> ()
            n1342 = local write "G#"(w237) -> ()
            n1343 = local write "C#"(w237) -> ()
            n1344 = local write "D"(w237) -> ()
            n1345 = local write "D#"(w237) -> ()
            n1346 = local write "E"(w237) -> ()
            n1347 = local write "A"(w237) -> ()
            n1348 = local write "A#"(w237) -> ()
            n1349 = local write "B"(w237) -> ()
            n1350 = local write "C"(w237) -> ()
          }
          frame 504..587 {
            w239 = FALSE
            n1351 = local write "F#"(TRUE) -> ()
            n1352 = local write "STANDBY"(w239) -> ()
            n1353 = local write "F"(w239) -> ()
            n1354 = local write "G"(w239) -> ()
            n1355 = local write "G#"(w239) -> ()
            n1356 = local write "C#"(w239) -> ()
            n1357 = local write "D"(w239) -> ()
            n1358 = local write "D#"(w239) -> ()
            n1359 = local write "E"(w239) -> ()
            n1360 = local write "A"(w239) -> ()
            n1361 = local write "A#"(w239) -> ()
            n1362 = local write "B"(w239) -> ()
            n1363 = local write "C"(w239) -> ()
          }
          frame 588..671 {
            w241 = FALSE
            n1364 = local write "G"(TRUE) -> ()
            n1365 = local write "STANDBY"(w241) -> ()
            n1366 = local write "F"(w241) -> ()
            n1367 = local write "F#"(w241) -> ()
            n1368 = local write "G#"(w241) -> ()
            n1369 = local write "C#"(w241) -> ()
            n1370 = local write "D"(w241) -> ()
            n1371 = local write "D#"(w241) -> ()
            n1372 = local write "E"(w241) -> ()
            n1373 = local write "A"(w241) -> ()
            n1374 = local write "A#"(w241) -> ()
            n1375 = local write "B"(w241) -> ()
            n1376 = local write "C"(w241) -> ()
          }
          frame 672..755 {
            w243 = FALSE
            n1377 = local write "G#"(TRUE) -> ()
            n1378 = local write "STANDBY"(w243) -> ()
            n1379 = local write "F"(w243) -> ()
            n1380 = local write "F#"(w243) -> ()
            n1381 = local write "G"(w243) -> ()
            n1382 = local write "C#"(w243) -> ()
            n1383 = local write "D"(w243) -> ()
            n1384 = local write "D#"(w243) -> ()
            n1385 = local write "E"(w243) -> ()
            n1386 = local write "A"(w243) -> ()
            n1387 = local write "A#"(w243) -> ()
            n1388 = local write "B"(w243) -> ()
            n1389 = local write "C"(w243) -> ()
          }
          frame 756..839 {
            w245 = FALSE
            n1390 = local write "A"(TRUE) -> ()
            n1391 = local write "F"(w245) -> ()
            n1392 = local write "F#"(w245) -> ()
            n1393 = local write "G"(w245) -> ()
            n1394 = local write "G#"(w245) -> ()
            n1395 = local write "C#"(w245) -> ()
            n1396 = local write "D"(w245) -> ()
            n1397 = local write "D#"(w245) -> ()
            n1398 = local write "E"(w245) -> ()
            n1399 = local write "STANDBY"(w245) -> ()
            n1400 = local write "A#"(w245) -> ()
            n1401 = local write "B"(w245) -> ()
            n1402 = local write "C"(w245) -> ()
          }
          frame 840..923 {
            w247 = FALSE
            n1403 = local write "A#"(TRUE) -> ()
            n1404 = local write "F"(w247) -> ()
            n1405 = local write "F#"(w247) -> ()
            n1406 = local write "G"(w247) -> ()
            n1407 = local write "G#"(w247) -> ()
            n1408 = local write "C#"(w247) -> ()
            n1409 = local write "D"(w247) -> ()
            n1410 = local write "D#"(w247) -> ()
            n1411 = local write "E"(w247) -> ()
            n1412 = local write "STANDBY"(w247) -> ()
            n1413 = local write "A"(w247) -> ()
            n1414 = local write "B"(w247) -> ()
            n1415 = local write "C"(w247) -> ()
          }
          frame 924..1000 {
            w249 = FALSE
            n1416 = local write "B"(TRUE) -> ()
            n1417 = local write "F"(w249) -> ()
            n1418 = local write "F#"(w249) -> ()
            n1419 = local write "G"(w249) -> ()
            n1420 = local write "G#"(w249) -> ()
            n1421 = local write "C#"(w249) -> ()
            n1422 = local write "D"(w249) -> ()
            n1423 = local write "D#"(w249) -> ()
            n1424 = local write "E"(w249) -> ()
            n1425 = local write "STANDBY"(w249) -> ()
            n1426 = local write "A"(w249) -> ()
            n1427 = local write "A#"(w249) -> ()
            n1428 = local write "C"(w249) -> ()
          }
        }
        n1429 = local write "Octave 7"(TRUE) -> ()
        n1430 = local write "Octave 3"(w222) -> ()
        n1431 = local write "Octave 2"(w222) -> ()
        n1432 = local write "Octave 1"(w222) -> ()
        n1433 = local write "Octave 0"(w222) -> ()
        n1434 = local write "Octave 4"(w222) -> ()
        n1435 = local write "Octave 8"(w222) -> ()
        n1436 = local write "Octave 6"(w222) -> ()
        n1437 = local write "Octave 5"(w222) -> ()
      }
      frame 225..255 {
        w251 = FALSE
        n1438 = case shown="0, Default" w253 {
          frame 0, Default {
            w254 = FALSE
            n1439 = local write "STANDBY"(TRUE) -> ()
            n1440 = local write "F"(w254) -> ()
            n1441 = local write "F#"(w254) -> ()
            n1442 = local write "G"(w254) -> ()
            n1443 = local write "G#"(w254) -> ()
            n1444 = local write "C#"(w254) -> ()
            n1445 = local write "D"(w254) -> ()
            n1446 = local write "D#"(w254) -> ()
            n1447 = local write "E"(w254) -> ()
            n1448 = local write "A"(w254) -> ()
            n1449 = local write "A#"(w254) -> ()
            n1450 = local write "B"(w254) -> ()
            n1451 = local write "C"(w254) -> ()
          }
          frame 1..83 {
            w256 = FALSE
            n1452 = local write "C"(TRUE) -> ()
            n1453 = local write "F"(w256) -> ()
            n1454 = local write "F#"(w256) -> ()
            n1455 = local write "G"(w256) -> ()
            n1456 = local write "G#"(w256) -> ()
            n1457 = local write "C#"(w256) -> ()
            n1458 = local write "D"(w256) -> ()
            n1459 = local write "D#"(w256) -> ()
            n1460 = local write "E"(w256) -> ()
            n1461 = local write "STANDBY"(w256) -> ()
            n1462 = local write "A"(w256) -> ()
            n1463 = local write "A#"(w256) -> ()
            n1464 = local write "B"(w256) -> ()
          }
          frame 84..167 {
            w258 = FALSE
            n1465 = local write "C#"(TRUE) -> ()
            n1466 = local write "F"(w258) -> ()
            n1467 = local write "F#"(w258) -> ()
            n1468 = local write "G"(w258) -> ()
            n1469 = local write "G#"(w258) -> ()
            n1470 = local write "STANDBY"(w258) -> ()
            n1471 = local write "D"(w258) -> ()
            n1472 = local write "D#"(w258) -> ()
            n1473 = local write "E"(w258) -> ()
            n1474 = local write "A"(w258) -> ()
            n1475 = local write "A#"(w258) -> ()
            n1476 = local write "B"(w258) -> ()
            n1477 = local write "C"(w258) -> ()
          }
          frame 168..251 {
            w260 = FALSE
            n1478 = local write "D"(TRUE) -> ()
            n1479 = local write "F"(w260) -> ()
            n1480 = local write "F#"(w260) -> ()
            n1481 = local write "G"(w260) -> ()
            n1482 = local write "G#"(w260) -> ()
            n1483 = local write "STANDBY"(w260) -> ()
            n1484 = local write "C#"(w260) -> ()
            n1485 = local write "D#"(w260) -> ()
            n1486 = local write "E"(w260) -> ()
            n1487 = local write "A"(w260) -> ()
            n1488 = local write "A#"(w260) -> ()
            n1489 = local write "B"(w260) -> ()
            n1490 = local write "C"(w260) -> ()
          }
          frame 252..335 {
            w262 = FALSE
            n1491 = local write "D#"(TRUE) -> ()
            n1492 = local write "F"(w262) -> ()
            n1493 = local write "F#"(w262) -> ()
            n1494 = local write "G"(w262) -> ()
            n1495 = local write "G#"(w262) -> ()
            n1496 = local write "STANDBY"(w262) -> ()
            n1497 = local write "C#"(w262) -> ()
            n1498 = local write "D"(w262) -> ()
            n1499 = local write "E"(w262) -> ()
            n1500 = local write "A"(w262) -> ()
            n1501 = local write "A#"(w262) -> ()
            n1502 = local write "B"(w262) -> ()
            n1503 = local write "C"(w262) -> ()
          }
          frame 336..419 {
            w264 = FALSE
            n1504 = local write "E"(TRUE) -> ()
            n1505 = local write "F"(w264) -> ()
            n1506 = local write "F#"(w264) -> ()
            n1507 = local write "G"(w264) -> ()
            n1508 = local write "G#"(w264) -> ()
            n1509 = local write "STANDBY"(w264) -> ()
            n1510 = local write "C#"(w264) -> ()
            n1511 = local write "D"(w264) -> ()
            n1512 = local write "D#"(w264) -> ()
            n1513 = local write "A"(w264) -> ()
            n1514 = local write "A#"(w264) -> ()
            n1515 = local write "B"(w264) -> ()
            n1516 = local write "C"(w264) -> ()
          }
          frame 420..503 {
            w266 = FALSE
            n1517 = local write "F"(TRUE) -> ()
            n1518 = local write "STANDBY"(w266) -> ()
            n1519 = local write "F#"(w266) -> ()
            n1520 = local write "G"(w266) -> ()
            n1521 = local write "G#"(w266) -> ()
            n1522 = local write "C#"(w266) -> ()
            n1523 = local write "D"(w266) -> ()
            n1524 = local write "D#"(w266) -> ()
            n1525 = local write "E"(w266) -> ()
            n1526 = local write "A"(w266) -> ()
            n1527 = local write "A#"(w266) -> ()
            n1528 = local write "B"(w266) -> ()
            n1529 = local write "C"(w266) -> ()
          }
          frame 504..587 {
            w268 = FALSE
            n1530 = local write "F#"(TRUE) -> ()
            n1531 = local write "STANDBY"(w268) -> ()
            n1532 = local write "F"(w268) -> ()
            n1533 = local write "G"(w268) -> ()
            n1534 = local write "G#"(w268) -> ()
            n1535 = local write "C#"(w268) -> ()
            n1536 = local write "D"(w268) -> ()
            n1537 = local write "D#"(w268) -> ()
            n1538 = local write "E"(w268) -> ()
            n1539 = local write "A"(w268) -> ()
            n1540 = local write "A#"(w268) -> ()
            n1541 = local write "B"(w268) -> ()
            n1542 = local write "C"(w268) -> ()
          }
          frame 588..671 {
            w270 = FALSE
            n1543 = local write "G"(TRUE) -> ()
            n1544 = local write "STANDBY"(w270) -> ()
            n1545 = local write "F"(w270) -> ()
            n1546 = local write "F#"(w270) -> ()
            n1547 = local write "G#"(w270) -> ()
            n1548 = local write "C#"(w270) -> ()
            n1549 = local write "D"(w270) -> ()
            n1550 = local write "D#"(w270) -> ()
            n1551 = local write "E"(w270) -> ()
            n1552 = local write "A"(w270) -> ()
            n1553 = local write "A#"(w270) -> ()
            n1554 = local write "B"(w270) -> ()
            n1555 = local write "C"(w270) -> ()
          }
          frame 672..755 {
            w272 = FALSE
            n1556 = local write "G#"(TRUE) -> ()
            n1557 = local write "STANDBY"(w272) -> ()
            n1558 = local write "F"(w272) -> ()
            n1559 = local write "F#"(w272) -> ()
            n1560 = local write "G"(w272) -> ()
            n1561 = local write "C#"(w272) -> ()
            n1562 = local write "D"(w272) -> ()
            n1563 = local write "D#"(w272) -> ()
            n1564 = local write "E"(w272) -> ()
            n1565 = local write "A"(w272) -> ()
            n1566 = local write "A#"(w272) -> ()
            n1567 = local write "B"(w272) -> ()
            n1568 = local write "C"(w272) -> ()
          }
          frame 756..839 {
            w274 = FALSE
            n1569 = local write "A"(TRUE) -> ()
            n1570 = local write "F"(w274) -> ()
            n1571 = local write "F#"(w274) -> ()
            n1572 = local write "G"(w274) -> ()
            n1573 = local write "G#"(w274) -> ()
            n1574 = local write "C#"(w274) -> ()
            n1575 = local write "D"(w274) -> ()
            n1576 = local write "D#"(w274) -> ()
            n1577 = local write "E"(w274) -> ()
            n1578 = local write "STANDBY"(w274) -> ()
            n1579 = local write "A#"(w274) -> ()
            n1580 = local write "B"(w274) -> ()
            n1581 = local write "C"(w274) -> ()
          }
          frame 840..923 {
            w276 = FALSE
            n1582 = local write "A#"(TRUE) -> ()
            n1583 = local write "F"(w276) -> ()
            n1584 = local write "F#"(w276) -> ()
            n1585 = local write "G"(w276) -> ()
            n1586 = local write "G#"(w276) -> ()
            n1587 = local write "C#"(w276) -> ()
            n1588 = local write "D"(w276) -> ()
            n1589 = local write "D#"(w276) -> ()
            n1590 = local write "E"(w276) -> ()
            n1591 = local write "STANDBY"(w276) -> ()
            n1592 = local write "A"(w276) -> ()
            n1593 = local write "B"(w276) -> ()
            n1594 = local write "C"(w276) -> ()
          }
          frame 924..1000 {
            w278 = FALSE
            n1595 = local write "B"(TRUE) -> ()
            n1596 = local write "F"(w278) -> ()
            n1597 = local write "F#"(w278) -> ()
            n1598 = local write "G"(w278) -> ()
            n1599 = local write "G#"(w278) -> ()
            n1600 = local write "C#"(w278) -> ()
            n1601 = local write "D"(w278) -> ()
            n1602 = local write "D#"(w278) -> ()
            n1603 = local write "E"(w278) -> ()
            n1604 = local write "STANDBY"(w278) -> ()
            n1605 = local write "A"(w278) -> ()
            n1606 = local write "A#"(w278) -> ()
            n1607 = local write "C"(w278) -> ()
          }
        }
        n1608 = local write "Octave 8"(TRUE) -> ()
        n1609 = local write "Octave 3"(w251) -> ()
        n1610 = local write "Octave 2"(w251) -> ()
        n1611 = local write "Octave 1"(w251) -> ()
        n1612 = local write "Octave 0"(w251) -> ()
        n1613 = local write "Octave 4"(w251) -> ()
        n1614 = local write "Octave 7"(w251) -> ()
        n1615 = local write "Octave 6"(w251) -> ()
        n1616 = local write "Octave 5"(w251) -> ()
      }
    }
    n1617 = Multiply(x=w7, y=8.0) -> (x*y=→"Frequency":dbl)
  }
  n1618 = VISA Close(VISA resource name=w4, error in (no error)=w5) -> ()  [unwired: 1 out]
